vi "Pane Size.vi"(8 "error in (no error)":errorcluster, 11 "2DArrayManager in":refnum<class "2DArrayManager.lvclass">) -> (0 "error out":errorcluster, 3 "2DArrayManager out":refnum<class "2DArrayManager.lvclass">)   [LabVIEW 2020, in "OOPanel.lvlib" / "2DArrayManager.lvclass"]
uses:
  2DArrayManager.lvclass
  2DArrayManager.lvclass/2DArrayManager.ctl
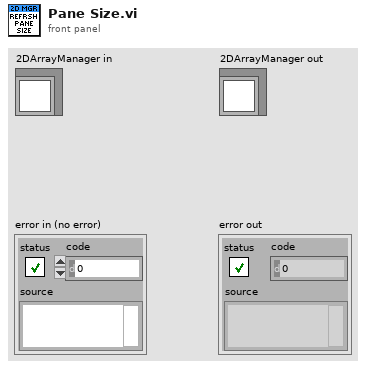
[diagram p1: front panel]
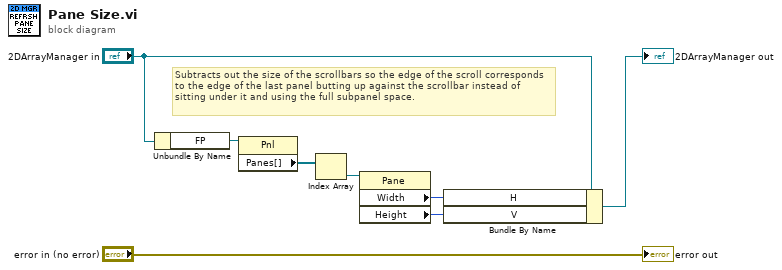
[diagram p0: block diagram]
diagram:
  # "Subtracts out the size of the scrollbars so the edge of the scroll corresponds to the edge of the last panel butting up against the scrollbar instead of sitting under it and using the full subpanel space."
  n1 = Unbundle By Name("2DArrayManager in") -> ("FP"=w4:refnum<vi>)
  n2 = property class="Pnl"(reference=w4) -> ("Panes[]"=w6:refnum<vi>[])  [unwired: 1 in, 2 out]
  n3 = Index Array(array=w6) -> (element=w5:refnum<vi>)  [unwired: 1 in]
  n4 = property class="Pane"(reference=w5) -> ("Width"=w2:u32, "Height"=w1:u32)  [unwired: 1 in, 2 out]
  n5 = Bundle By Name(cluster="2DArrayManager in", "H"=w2, "V"=w1) -> (→"2DArrayManager out":refnum<class "2DArrayManager.lvclass">)
  "error out" <- "error in (no error)"
